vi "Dlg_Graph.vi"(0 "Channels":T1(array[cluster]), 11 "error in":errorcluster) -> (15 "error out":errorcluster)   [LabVIEW 2026]
doc: "그래프 팝업 창(1300x720): AIDAQ_GRAPH 큐의 최신 데이터를 100 ms마다 그림. 닫기 버튼이나 창 닫기로 종료."
panel:
  in  "닫기":bool
  out "Graph":picture
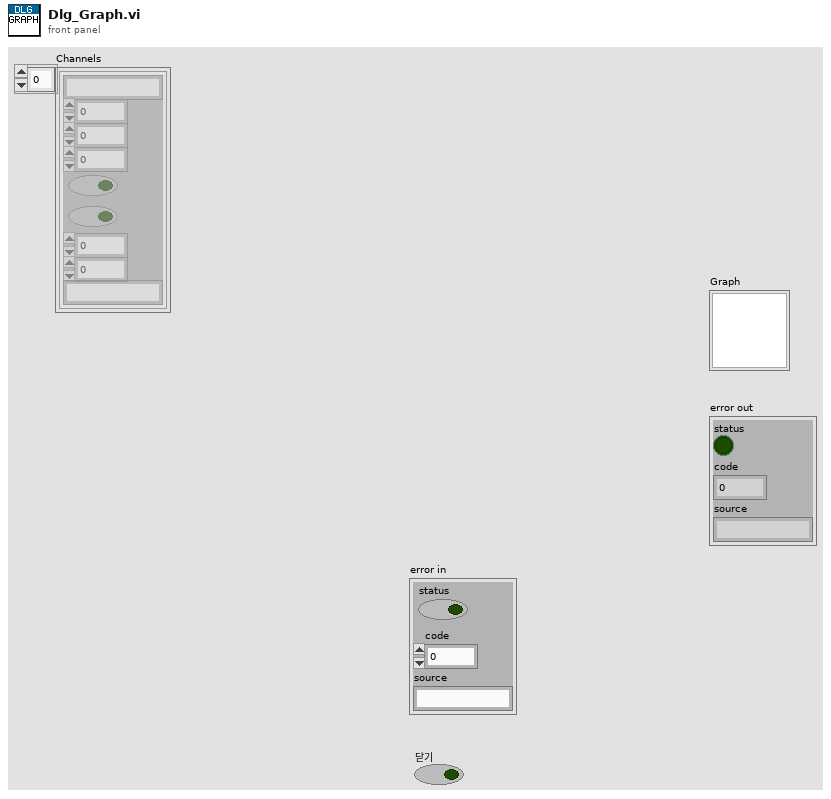
[diagram p1: front panel]
types:
  T1 = cluster{"Name":string, "Value":dbl, "High Limit":dbl, "Low Limit":dbl, "Save":bool, "Graph":bool, "Scale Min":dbl, "Scale Max":dbl, "Unit":string}[]
  T2 = cluster{"Data":dbl[][], "Values":dbl[], "dt":dbl, "Running":bool, "Logging":bool, "Message":string, "Log File":path}
  T3 = cluster{"Left":i32, "Top":i32, "Right":i32, "Bottom":i32}
  T4 = cluster{"left":i16, "top":i16, "right":i16, "bottom":i16}
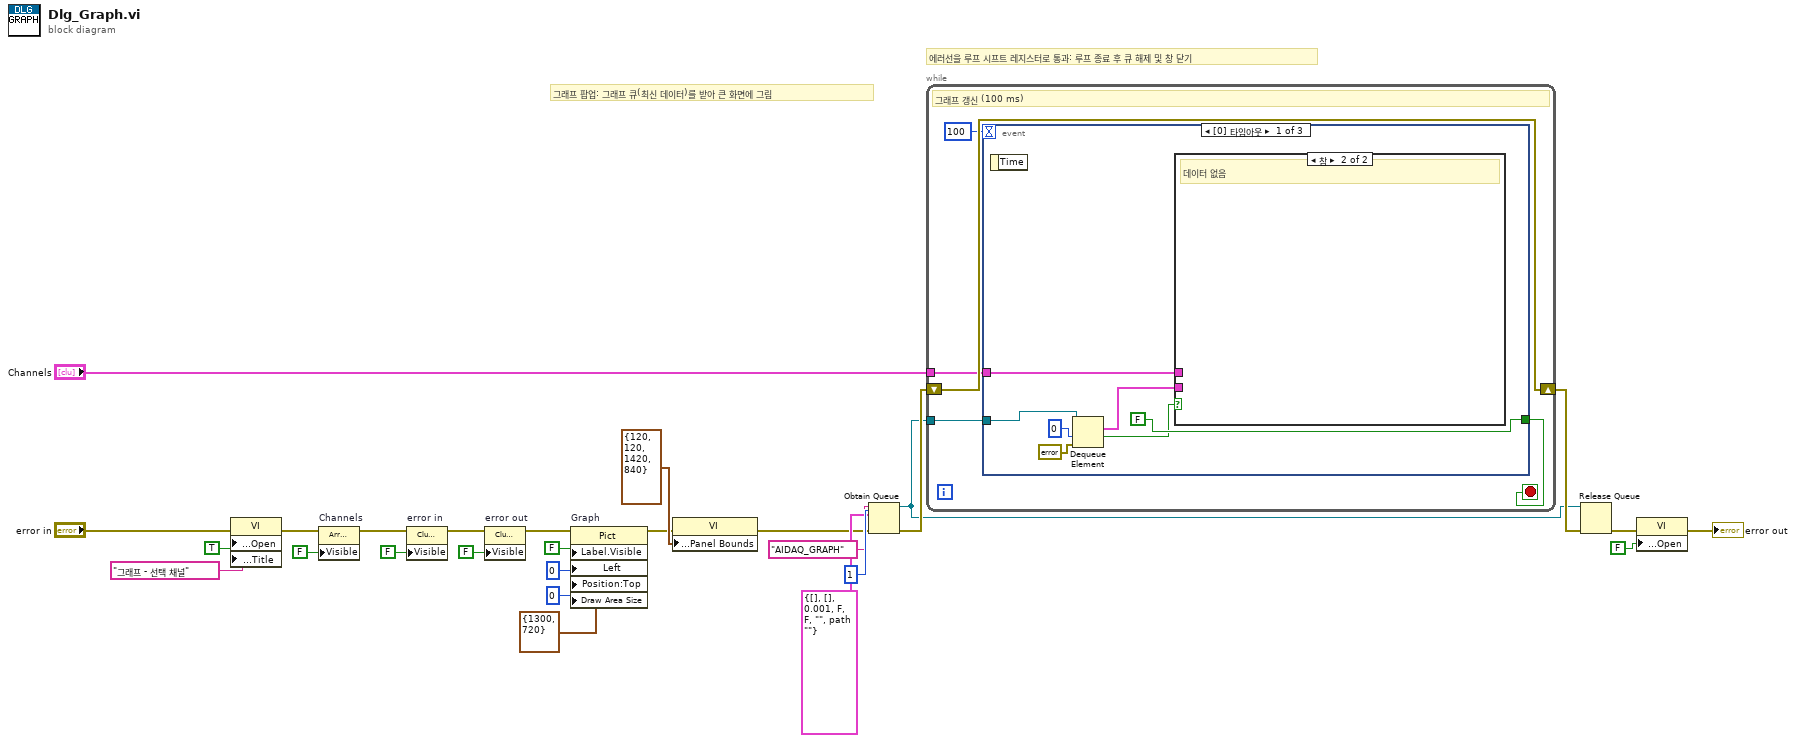
[diagram p0: block diagram]
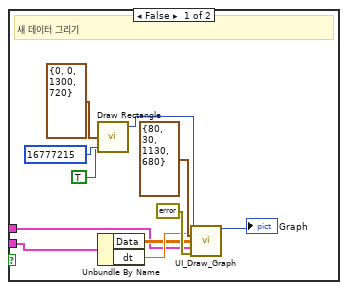
[diagram p2: hidden frame]
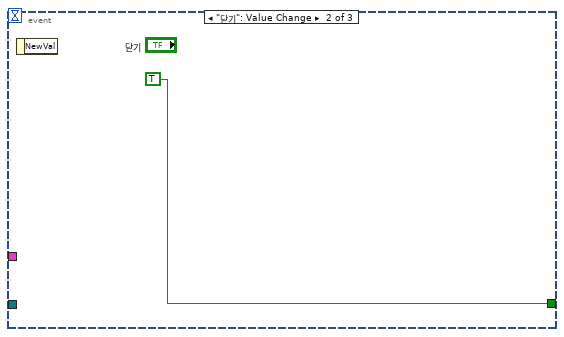
[diagram p3: hidden frame]
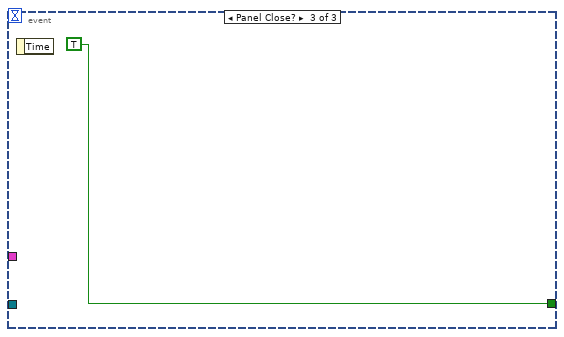
[diagram p4: hidden frame]
diagram:
  # "에러선을 루프 시프트 레지스터로 통과: 루프 종료 후 큐 해제 및 창 닫기"
  # "그래프 팝업: 그래프 큐(최신 데이터)를 받아 큰 화면에 그림"
  n1 = property class="VI"(error in="error in", "Front Panel Window:Open"=TRUE, "Front Panel Window:Title"="그래프 - 선택 채널") -> (error out=w5:errorcluster)  [unwired: 1 in, 1 out]
  n2 = property on="Channels" class="Arr (엄격한)"(error in=w5, "Visible"=FALSE) -> (error out=w7:errorcluster)  [unwired: 1 in, 1 out]
  n3 = property on="error in" class="Clust (엄격한)"(error in=w7, "Visible"=FALSE) -> (error out=w9:errorcluster)  [unwired: 1 in, 1 out]
  n4 = property on="error out" class="Clust (엄격한)"(error in=w9, "Visible"=FALSE) -> (error out=w11:errorcluster)  [unwired: 1 in, 1 out]
  n5 = property on="Graph" class="Pict"(error in=w11, "Label.Visible"=FALSE, "Left"=0, "Position:Top"=0, "Draw Area Size"=cluster{"Width":i32, "Height":i32} {"Width"=1300, "Height"=720}) -> (error out=w16:errorcluster)  [unwired: 1 in, 1 out]
  n6 = property class="VI"(error in=w16, "Front Panel Window:Panel Bounds"=T3 {"Left"=120, "Top"=120, "Right"=1420, "Bottom"=840}) -> (error out=w18:errorcluster)  [unwired: 1 in, 1 out]
  n7 = Obtain Queue(max queue size (-1, unlimited)=1, name (unnamed)="AIDAQ_GRAPH", element data type=T2 {"Data"=[], "Values"=[], "dt"=0.001, "Running"=FALSE, "Logging"=FALSE, "Message"="", "Log File"=path ""}, error in (no error)=w18) -> (queue out=w22:refnum<queue>, error out=w23:errorcluster)  [unwired: 1 in, 1 out]
  n8 = while {
    tunnel: "Channels" -> [w29]
    tunnel: w22 -> [w28]
    shift-right: [w32] -> w24
    shift-left: w23 -> [w32]
    stop <- w31 stop-if-true
    # "그래프 갱신 (100 ms)"
    n9 = event shown="[0] 타임아웃" {
      selector: _ -> [_ _ _]
      dyn-events: _ -> [_ _ _]
      timeout: 100 -> [_ _ _]
      tunnel: [FALSE TRUE TRUE] -> w31
      tunnel: w29 -> [w34 _ _]
      tunnel: w28 -> [w33 _ _]
      event Timeout {
        n10 = event-data() -> ()  [unwired: 1 in, 1 out]
        n11 = Dequeue Element(queue=w33, timeout in ms (-1)=0, error in (no error)=errorcluster {"status"=FALSE, "code"=0, "source"=""}) -> (element=w37:T2, timed out?=w38:bool)  [unwired: 2 out]
        n12 = case shown="참" w38 {
          tunnel: w34 -> [w41 _]
          tunnel: w37 -> [w40 _]
          frame False {
            # "새 데이터 그리기"
            n13 = call <vilib>:"Draw Rectangle.vi"("rect"=T4 {"left"=0, "top"=0, "right"=1300, "bottom"=720}, "fill?(F)"=TRUE, "color(black)"=u32 16777215) -> ("new picture"=w47:picture)  [unwired: 6 in]
            n14 = Unbundle By Name(w40) -> ("Data"=w42:dbl[][], "dt"=w43:dbl)
            n15 = call "UI_Draw_Graph.vi"("Picture"=w47, "dt"=w43, "Plot Rect"=T4 {"left"=80, "top"=30, "right"=1130, "bottom"=680}, "Data"=w42, "Channels"=w41, "error in"=errorcluster {"status"=FALSE, "code"=0, "source"=""}) -> ("New Picture"=→"Graph":picture)  [unwired: 8 in, 1 out]
          }
          frame True {
            # "데이터 없음"
          }
        }
      }
      event "닫기": Value Change {
        n16 = event-data() -> ()  [unwired: 1 in, 1 out]
      }
      event Panel Close? {
        n17 = event-data() -> ()  [unwired: 2 in, 1 out]
        n18 = event-data() -> ()  [unwired: 1 in, 1 out]
      }
    }
  }
  n19 = Release Queue(queue=w22, error in (no error)=w24) -> (error out=w25:errorcluster)  [unwired: 1 in, 2 out]
  n20 = property class="VI"(error in=w25, "Front Panel Window:Open"=FALSE) -> (error out=→"error out":errorcluster)  [unwired: 1 in, 1 out]
